vi "var to string (ring).vi"(10 "Ring Refnum":refnum<vi>, 11 "reference":refnum<vi>) -> (3 "ring text":string)   [LabVIEW 2025]
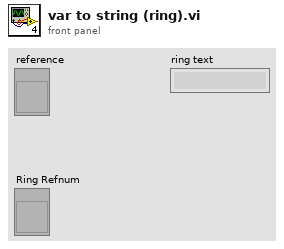
[diagram p1: front panel]
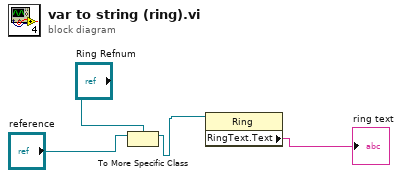
[diagram p0: block diagram]
diagram:
  n1 = To More Specific Class(target class="Ring Refnum", reference="reference") -> (specific class reference=w4:refnum<vi>)  [unwired: 1 in, 1 out]
  n2 = property class="Ring"(reference=w4) -> ("RingText.Text"=→"ring text":string)  [unwired: 1 in, 2 out]
